vi "Write configuration.vi"(8 "error in":errorcluster, 10 "configuration":refnum<class "NISE_CEF_serializable configuration.lvclass">, 11 "Systems in":refnum<class "Systems.lvclass">) -> (0 "error out":errorcluster, 3 "Systems out":refnum<class "Systems.lvclass">)   [LabVIEW 2013, in "PL Framework Configuration Tool.lvlib" / "Systems.lvclass"]
uses:
  Systems.lvclass
  <vilib>/NI/Configuration Framework/serializable configuration/NISE_CEF_serializable configuration.lvclass
  Framework Configuration Classes/system configuration/PL_System Configuration.lvclass
  Systems.lvclass/Systems.ctl
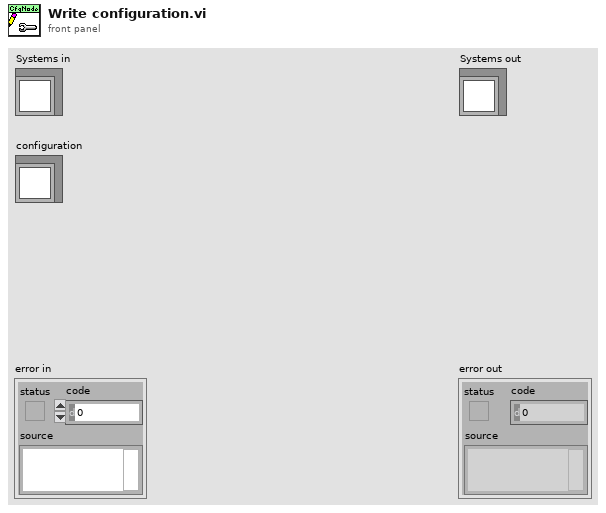
[diagram p1: front panel]
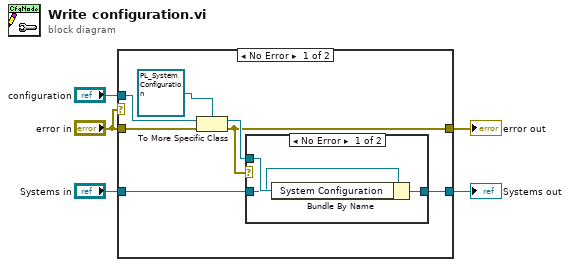
[diagram p0: block diagram]
diagram:
  n1 = case shown="No Error" "error in" {
    tunnel: "configuration" -> [w10 _]
    tunnel: [w9 w17] -> w4
    tunnel: "Systems in" -> [w8 w17]
    tunnel: "error in" -> [w7 w18]
    tunnel: [w6 w18] -> w2
    frame No Error {
      n2 = To More Specific Class(target class=refnum<class "PL_System Configuration.lvclass"> refnum ("System Configuration"), reference=w10, error in=w7) -> (specific class reference=w11:refnum<class "PL_System Configuration.lvclass">, error out=w6:errorcluster)
      n3 = case shown="No Error" w6 {
        tunnel: w11 -> [w15 _]
        tunnel: [w14 w16] -> w9
        tunnel: w8 -> [w13 w16]
        frame No Error {
          n4 = Bundle By Name(cluster=w13, "System Configuration"=w15) -> (w14:refnum<class "Systems.lvclass">)
        }
        frame Error {
        }
      }
    }
    frame Error {
    }
  }
  "error out" <- w2
  "Systems out" <- w4
